vi "FlatToRichcif_can_reader_cansub_CansubDevice.vi"(5 "OutputClusterType":T1, 11 "InputCluster":T2) -> (3 "OutputCluster":T1)   [LabVIEW 2021, in "CanReaderCansub_client.lvlib"]
uses:
  CanReaderCansub_client.lvlib
  cif_can_reader_cansub_CansubDevice_Flat.ctl
  cif_can_reader_cansub_CansubDevice.ctl
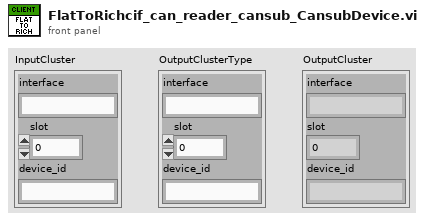
[diagram p1: front panel]
types:
  T1 = typedef "CanReaderCansub_client.lvlib/cif_can_reader_cansub_CansubDevice.ctl" = cluster{"interface":string, "slot":u32, "device_id":string}
  T2 = typedef "CanReaderCansub_client.lvlib/cif_can_reader_cansub_CansubDevice_Flat.ctl" = cluster{"interface":string, "slot":u32, "device_id":string}
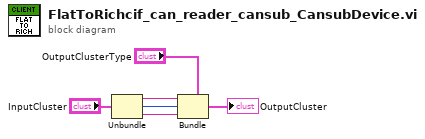
[diagram p0: block diagram]
diagram:
  n1 = Unbundle "Unbundle"("InputCluster") -> ("interface"=w3:string, "slot"=w2:u32, "device_id"=w1:string)
  n2 = Bundle "Bundle"(cluster="OutputClusterType", "interface"=w3, "slot"=w2, "device_id"=w1) -> (→"OutputCluster":T1)
